vi "New.vi"(11 "age limit (1)[days]":dbl=1.0) -> (3 "RolloverTrigger.Age":refnum<class "RolloverTrigger.Age.lvclass">)   [LabVIEW 2018, in "GLog.lvlib" / "RolloverTrigger.Age.lvclass"]
uses:
  RolloverTrigger.Age.lvclass
  RolloverTrigger.Age.lvclass/RolloverTrigger.Age.ctl
panel:
  # "Connector Pane"
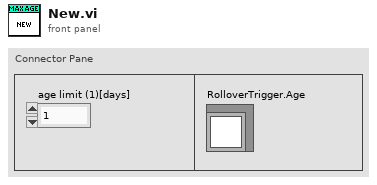
[diagram p1: front panel]
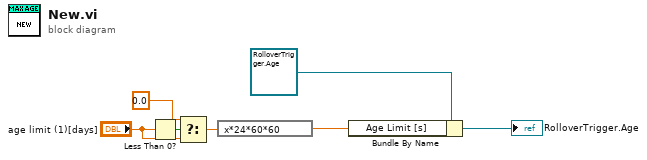
[diagram p0: block diagram]
diagram:
  n1 = Less Than 0?(x="age limit (1)[days]") -> (x < 0?=w4:bool)
  n2 = Select(t=0.0, s=w4, f="age limit (1)[days]") -> (s? t:f=w1:dbl)
  n3 = expression code="x*24*60*60"(w1) -> (w6:dbl)
  n4 = Bundle By Name(cluster=refnum<class "RolloverTrigger.Age.lvclass"> refnum ("RolloverTrigger.Age out"), "Age Limit [s]"=w6) -> (→"RolloverTrigger.Age":refnum<class "RolloverTrigger.Age.lvclass">)
